vi "Queue-Push Multiple Elements.vi"(8 "error in":errorcluster, 10 "elements":variant[](array[variant]), 11 "Buffer in":refnum<data-value>) -> (0 "error out":errorcluster, 2 "overflow":variant[](array[variant]), 3 "Buffer":refnum<data-value>)   [LabVIEW 2013, in "CircularBuffer.lvlib" / "VariantBuffer.lvclass"]
doc: "This VI allows to input an array into the buffer. The location in the buffer is updated automatically.\n\nIf the input array is larger than the buffer then just take last elements of the input array and save them in the buffer. Also give a warning that this happened."
uses:
  VariantBuffer.lvclass
  buffer-errors -- ring.ctl
  VariantBuffer.lvclass/VariantBuffer.ctl
  buffer-event -- enum.ctl
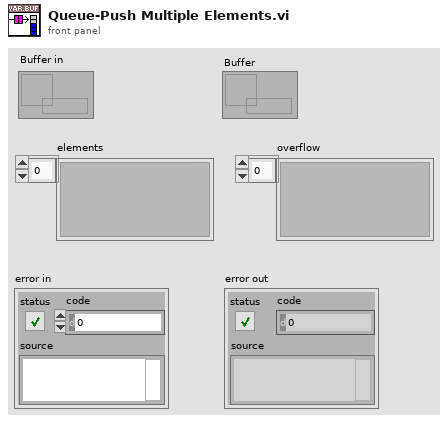
[diagram p1: front panel]
types:
  T1 = typedef "CircularBuffer.lvlib/VariantBuffer.lvclass/buffer-errors -- ring.ctl" = i32
  T2 = typedef "CircularBuffer.lvlib/VariantBuffer.lvclass/buffer-type -- enum.ctl" = enum16{"Queue", "Stack"}
  T3 = typedef "CircularBuffer.lvlib/VariantBuffer.lvclass/buffer-event -- enum.ctl" = enum16{"element-added", "element-removed", "filled", "emptied", "resized", "default-changed", "destroyed"}
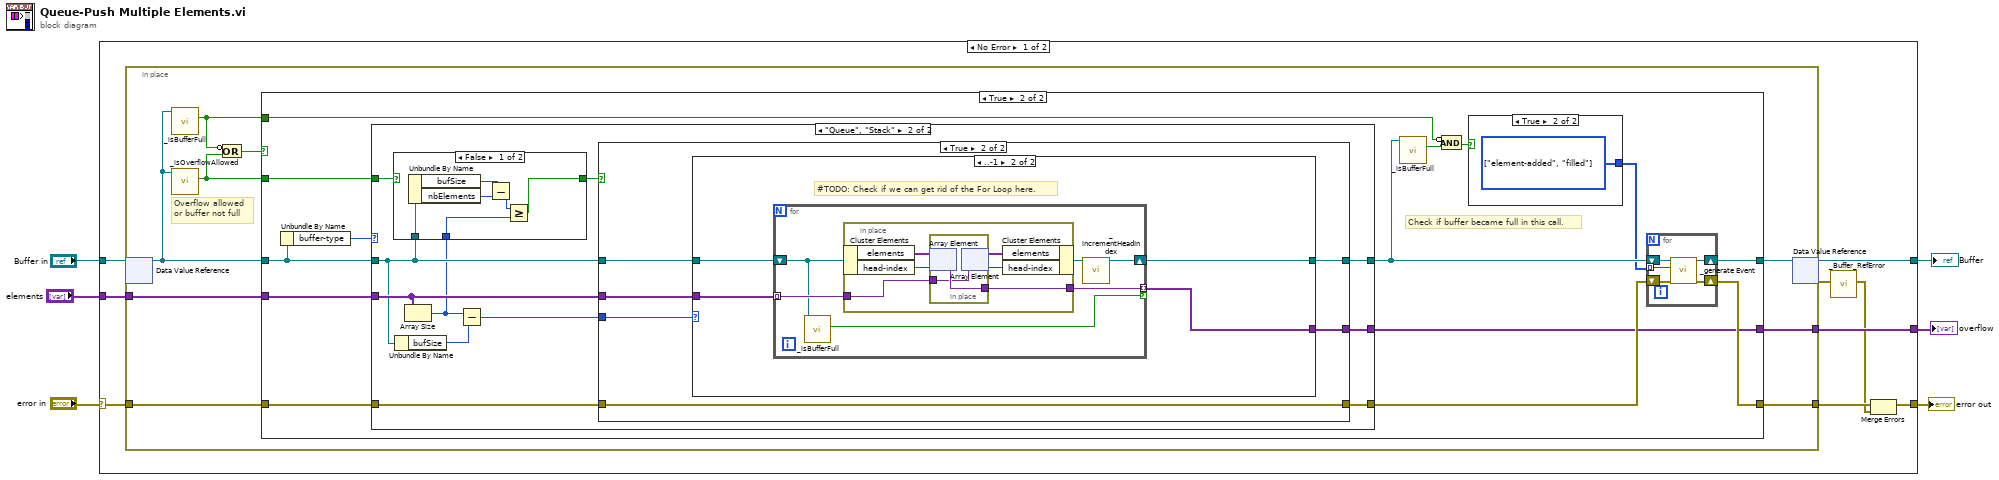
[diagram p0: block diagram]
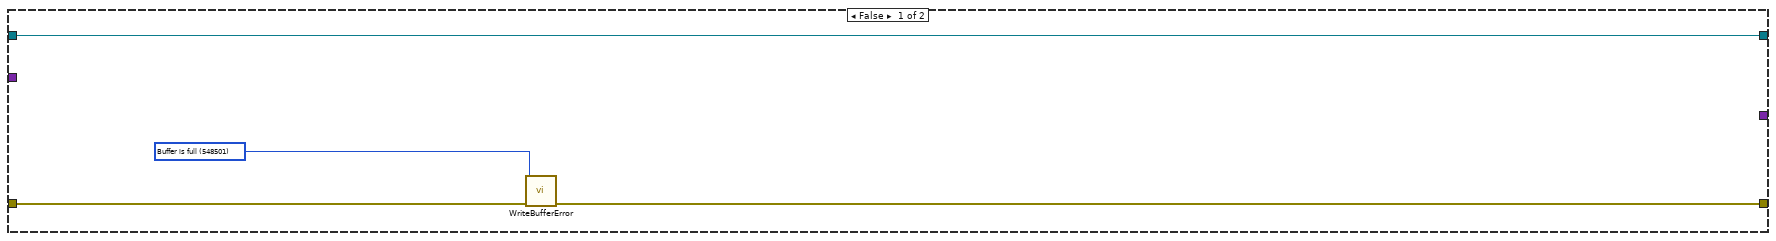
[diagram p2: hidden frame]
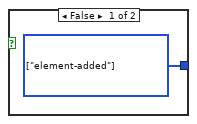
[diagram p3: hidden frame]
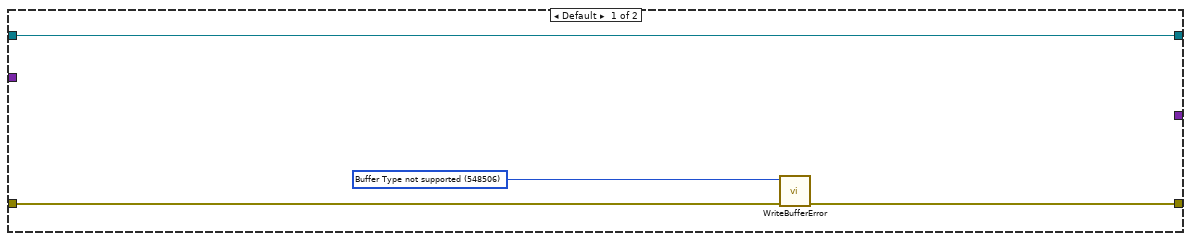
[diagram p4: hidden frame]
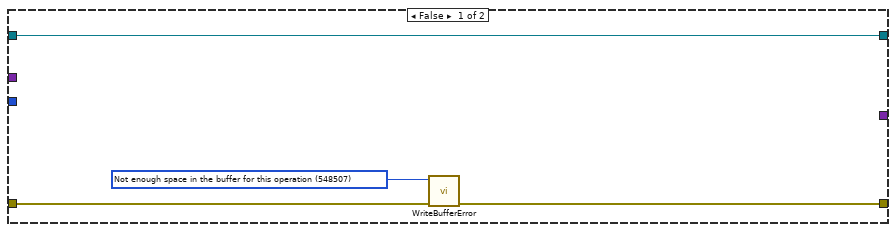
[diagram p5: hidden frame]
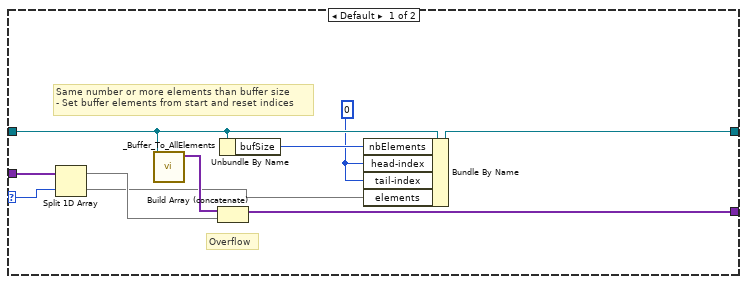
[diagram p6: hidden frame]
diagram:
  n1 = case shown="No Error" "error in" {
    selector: "error in" -> [w10 w111]
    tunnel: "Buffer in" -> [w15 w110]
    tunnel: [w12 w110] -> w5
    tunnel: [w14 w111] -> w4
    tunnel: "elements" -> [w13 _]
    tunnel: [w11 _] -> w1
    frame No Error {
      n2 = in-place {
        in-place-border: w13 -> [w24]
        in-place-border: [w23] -> w11
        in-place-border: w10 -> [w19]
        in-place-border: [w18] -> w9
        # "Overflow allowed\nor buffer not full"
        n3 = in-place-dvr #1(w15) -> (w22:refnum<class "VariantBuffer.lvclass">)  [unwired: 1 out]
        n4 = call "_isBufferFull.vi"("VariantBuffer in"=w22) -> ("isFull"=w17:bool)  [unwired: 10 in]
        n5 = call "_isOverflowAllowed.vi"("VariantBuffer in"=w22) -> ("Allow Overflow?"=w16:bool)  [unwired: 10 in]
        n6 = Compound Arithmetic op=OR(invert w17, w16) -> (w21:bool)
        n7 = case shown="True" w21 {
          tunnel: w24 -> [_ w31]
          tunnel: [w26 w40] -> w20
          tunnel: [_ w30] -> w23
          tunnel: w22 -> [w26 w32]
          tunnel: w19 -> [w28 w41]
          tunnel: [w27 w39] -> w18
          tunnel: w17 -> [_ w33]
          tunnel: w16 -> [_ w29]
          frame False {
            w25 = T1 548501 items=["No error"=0, "Generic Buffer error"=548500, "Buffer is full"=548501, "Buffer is empty"=548502, "Buffer size cannot be 0"=548503, "Buffer reference is invalid"=548504, "Buffer event reference invalid"=548505] ("buffer-errors")
            n8 = call "WriteBufferError.vi"("error in (no error)"=w28, "buffer-errors"=w25) -> ("error out"=w27:errorcluster)  [unwired: 9 in]
          }
          frame True {
            # "Check if buffer became full in this call."
            n9 = Unbundle By Name(w32) -> ("buffer-type"=w42:T2)
            n10 = case shown="\"Queue\", \"Stack\"" w42 {
              tunnel: w31 -> [_ w63]
              tunnel: [_ w62] -> w30
              tunnel: w32 -> [w53 w56]
              tunnel: [w53 w64] -> w37
              tunnel: [w51 w58] -> w38
              tunnel: w41 -> [w52 w57]
              tunnel: w29 -> [_ w60]
              frame Default {
                w50 = T1 548506 items=["No error"=0, "Generic Buffer error"=548500, "Buffer is full"=548501, "Buffer is empty"=548502, "Buffer size cannot be 0"=548503, "Buffer reference is invalid"=548504, "Buffer event reference invalid"=548505, "Buffer Type not supported"=548506] ("buffer-errors")
                n11 = call "WriteBufferError.vi"("error in (no error)"=w52, "buffer-errors"=w50) -> ("error out"=w51:errorcluster)  [unwired: 9 in]
              }
              frame "Queue", "Stack" {
                n12 = Unbundle By Name(w56) -> ("bufSize"=w61:i32)
                n13 = Array Size(array=w63) -> (size(s)=w55:i32)
                n14 = case shown="False" w60 {
                  selector: w60 -> [_ w109]
                  tunnel: [w103 w109] -> w59
                  tunnel: w56 -> [w108 _]
                  tunnel: w55 -> [w104 _]
                  frame False {
                    n15 = Unbundle By Name(w108) -> ("bufSize"=w107:i32, "nbElements"=w106:i32)
                    n16 = Subtract(x=w107, y=w106) -> (x-y=w105:i32)
                    n17 = Greater Or Equal?(x=w105, y=w104) -> (x >= y?=w103:bool)
                  }
                  frame True {
                  }
                }
                n18 = Subtract(x=w55, y=w61) -> (x-y=w54:i32)
                n19 = case shown="True" w59 {
                  tunnel: [w66 w74] -> w64
                  tunnel: w63 -> [_ w69]
                  tunnel: [_ w73] -> w62
                  tunnel: w56 -> [w66 w72]
                  tunnel: w54 -> [_ w71]
                  tunnel: [w67 w70] -> w58
                  tunnel: w57 -> [w68 w70]
                  frame False {
                    w65 = T1 548507 items=["No error"=0, "Generic Buffer error"=548500, "Buffer is full"=548501, "Buffer is empty"=548502, "Buffer size cannot be 0"=548503, "Buffer reference is invalid"=548504, "Buffer event reference invalid"=548505, "Buffer Type not supported"=548506, "Not enough space in the buffer for this operation"=548507] ("buffer-errors")
                    n20 = call "WriteBufferError.vi"("error in (no error)"=w68, "buffer-errors"=w65) -> ("error out"=w67:errorcluster)  [unwired: 9 in]
                  }
                  frame True {
                    n21 = case shown="..-1" w71 {
                      selector: w71 -> [w77 _]
                      tunnel: [w84 w86] -> w74
                      tunnel: w72 -> [w83 w88]
                      tunnel: [w82 w85] -> w73
                      tunnel: w69 -> [w78 w87]
                      frame Default {
                        w80 = 0 ("head-index")
                        # "Overflow"
                        # "Same number or more elements than buffer size\n- Set buffer elements from start and reset indices"
                        n22 = Split 1D Array(array=w78, index=w77) -> (first subarray=w76:variant[], second subarray=w75:variant[])
                        n23 = call "_Buffer_To_AllElements.vi"("Buffer"=w83) -> ("elements"=w79:variant[])  [unwired: 10 in]
                        n24 = Build Array (concatenate)(w79, w76) -> (w82:variant[])
                        n25 = Unbundle By Name(w83) -> ("bufSize"=w81:i32)
                        n26 = Bundle By Name(cluster=w83, "nbElements"=w81, "head-index"=w80, "tail-index"=w80, "elements"=w75) -> (w84:refnum<class "VariantBuffer.lvclass">)
                      }
                      frame ..-1 {
                        # "#TODO: Check if we can get rid of the For Loop here."
                        n27 = for {
                          tunnel: w87 -> [w93] mode=indexing
                          shift-right: [w92] -> w86
                          shift-left: w88 -> [w91]
                          tunnel: [w90] -> w85 mode=indexing if=w89
                          n28 = call "_isBufferFull.vi"("VariantBuffer in"=w91) -> ("isFull"=w89:bool)  [unwired: 10 in]
                          n29 = in-place {
                            in-place-border: [w97] -> w90
                            in-place-border: w93 -> [w95]
                            n30 = in-place-cluster #2(w91) -> ("elements"=w100:variant[], "head-index"=w98:i32)
                            n31 = in-place {
                              in-place-border: w95 -> [w101]
                              in-place-border: [w102] -> w97
                              n32 = in-place-array #3(w100, w98) -> (w102:variant)
                              n33 = in-place-array #3(w101) -> (w99:variant[], w96:i32)
                            }
                            n34 = in-place-cluster #2("elements"=w99, "head-index"=w96) -> (w94:refnum<class "VariantBuffer.lvclass">)
                          }
                          n35 = call "_incrementHeadIndex.vi"("VariantBuffer in"=w94) -> ("VariantBuffer out"=w92:refnum<class "VariantBuffer.lvclass">)  [unwired: 10 in]
                        }
                      }
                    }
                  }
                }
              }
            }
            n36 = call "_isBufferFull.vi"("VariantBuffer in"=w37) -> ("isFull"=w36:bool)  [unwired: 10 in]
            n37 = Compound Arithmetic op=AND(invert w33, w36) -> (w35:bool)
            n38 = case shown="True" w35 {
              tunnel: [w43 w44] -> w34
              frame False {
                w43 = T3[] [enum."element-added"] items=["element-added", "element-removed", "filled", "emptied", "resized", "default-changed", "destroyed"]
              }
              frame True {
                w44 = T3[] [enum."element-added", enum."filled"] items=["element-added", "element-removed", "filled", "emptied", "resized", "default-changed", "destroyed"]
              }
            }
            n39 = for {
              tunnel: w34 -> [w47] mode=indexing
              shift-right: [w49] -> w40
              shift-left: w37 -> [w48]
              shift-right: [w46] -> w39
              shift-left: w38 -> [w45]
              n40 = call "_generate Event.vi"("error in"=w45, "event"=w47, "VariantBuffer"=w48) -> ("error out"=w46:errorcluster, "VariantBuffer out"=w49:refnum<class "VariantBuffer.lvclass">)  [unwired: 7 in]
            }
          }
        }
        n41 = in-place-dvr #1(w20) -> (w12:refnum<data-value>, w8:errorcluster)
      }
      n42 = call "_Buffer_RefError.vi"("error in (no error)"=w8) -> ("error out"=w7:errorcluster)  [unwired: 10 in]
      n43 = Merge Errors(w9, w7) -> (w14:errorcluster)
    }
    frame Error {
    }
  }
  "error out" <- w4
  "Buffer" <- w5
  "overflow" <- w1
